vi "DSS-Tests-run_param_vi.vi"(7 "increment temp":dbl=0.1, 8 "error in":errorcluster, 9 "stop temp":dbl=60.0, 10 "start temp":dbl=-5.0, 11 "vi relative path":string) -> (0 "error out":errorcluster, 3 "array variant":variant)   [LabVIEW 2020, in "DSS-Tests.lvlib"]
doc: "Runs a parameter-table VI by VI Server: opens it by path, sets Start temp, Stop Temp and Increment temp, runs it to the end and returns its Array indicator as a variant."
uses:
  DSS-Tests.lvlib
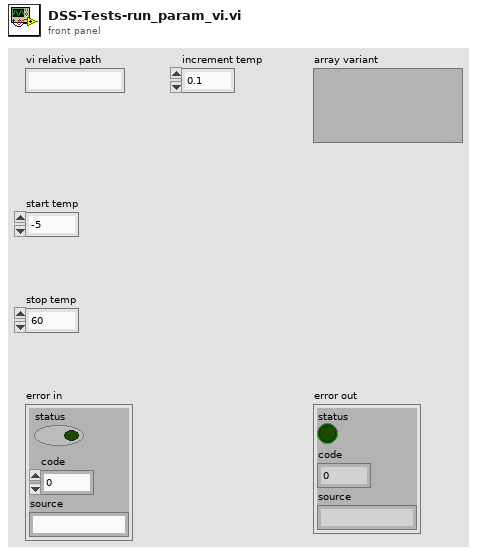
[diagram p1: front panel]
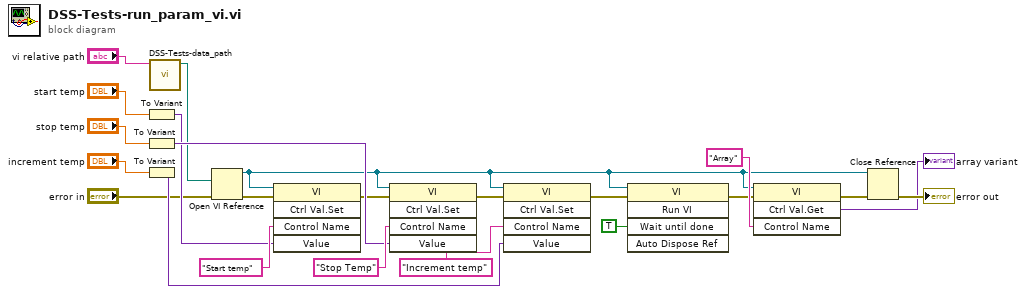
[diagram p0: block diagram]
diagram:
  n1 = To Variant(anything="start temp") -> (Variant=w9:variant)
  n2 = To Variant(anything="stop temp") -> (Variant=w12:variant)
  n3 = To Variant(anything="increment temp") -> (Variant=w15:variant)
  n4 = call "DSS-Tests-data_path.vi"("relative path"="vi relative path") -> ("path"=w6:path)  [unwired: 10 in]
  n5 = Open VI Reference(vi path=w6, error in (no error)="error in") -> (vi reference=w7:refnum<vi>, error out=w8:errorcluster)  [unwired: 4 in]
  n6 = invoke class="VI" method="Ctrl Val.Set"(reference=w7, error in=w8, "Control Name"="Start temp", "Value"=w9) -> (error out=w11:errorcluster)  [unwired: 1 in, 4 out]
  n7 = invoke class="VI" method="Ctrl Val.Set"(reference=w7, error in=w11, "Control Name"="Stop Temp", "Value"=w12) -> (error out=w14:errorcluster)  [unwired: 1 in, 4 out]
  n8 = invoke class="VI" method="Ctrl Val.Set"(reference=w7, error in=w14, "Control Name"="Increment temp", "Value"=w15) -> (error out=w17:errorcluster)  [unwired: 1 in, 4 out]
  n9 = invoke class="VI" method="Run VI"(reference=w7, error in=w17, "Wait until done"=TRUE) -> (error out=w19:errorcluster)  [unwired: 2 in, 4 out]
  n10 = invoke class="VI" method="Ctrl Val.Get"(reference=w7, error in=w19, "Control Name"="Array") -> (error out=w21:errorcluster, "Get Control Value Variant"=→"array variant":variant)  [unwired: 1 in, 2 out]
  n11 = Close Reference(reference=w7, error in (no error)=w21) -> (error out=→"error out":errorcluster)
